vi "test completion complete.vi"(8 "error in (no error)":errorcluster) -> (0 "error out":errorcluster, 3 "body":string)   [LabVIEW 2020, in "MCP Server tests.lvlib"]
doc: "completion/complete (MCP utility completion) in both eras. A legacy initialize (id 731) and a modern server/discover (id 732) declare capabilities.completions {}. completion/complete for the prompt fake_prompt_concatanate_strings is answered with completion.values [], total 0 and hasMore false, legacy (id 733) and modern (id 734, HTTP 200 with resultType complete). completion/complete for a prompt the server does not have (id 735) is answered with the JSON-RPC error -32602 and the request id. The requests are sent with the LabVIEW HTTP Client directly."
uses:
  MCP Server tests.lvlib
  <vilib>/addons/_JKI Toolkits/Caraya/classes/Test/Test.lvclass
  <vilib>/addons/_JKI Toolkits/Caraya/classes/Assert/Assert.lvclass
panel:
  out "lookup error":errorcluster
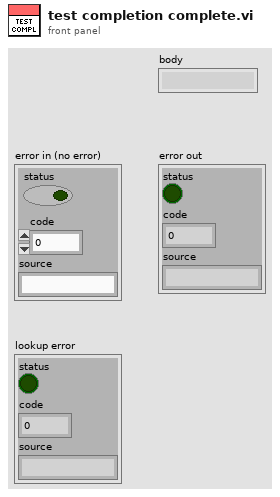
[diagram p1: front panel]
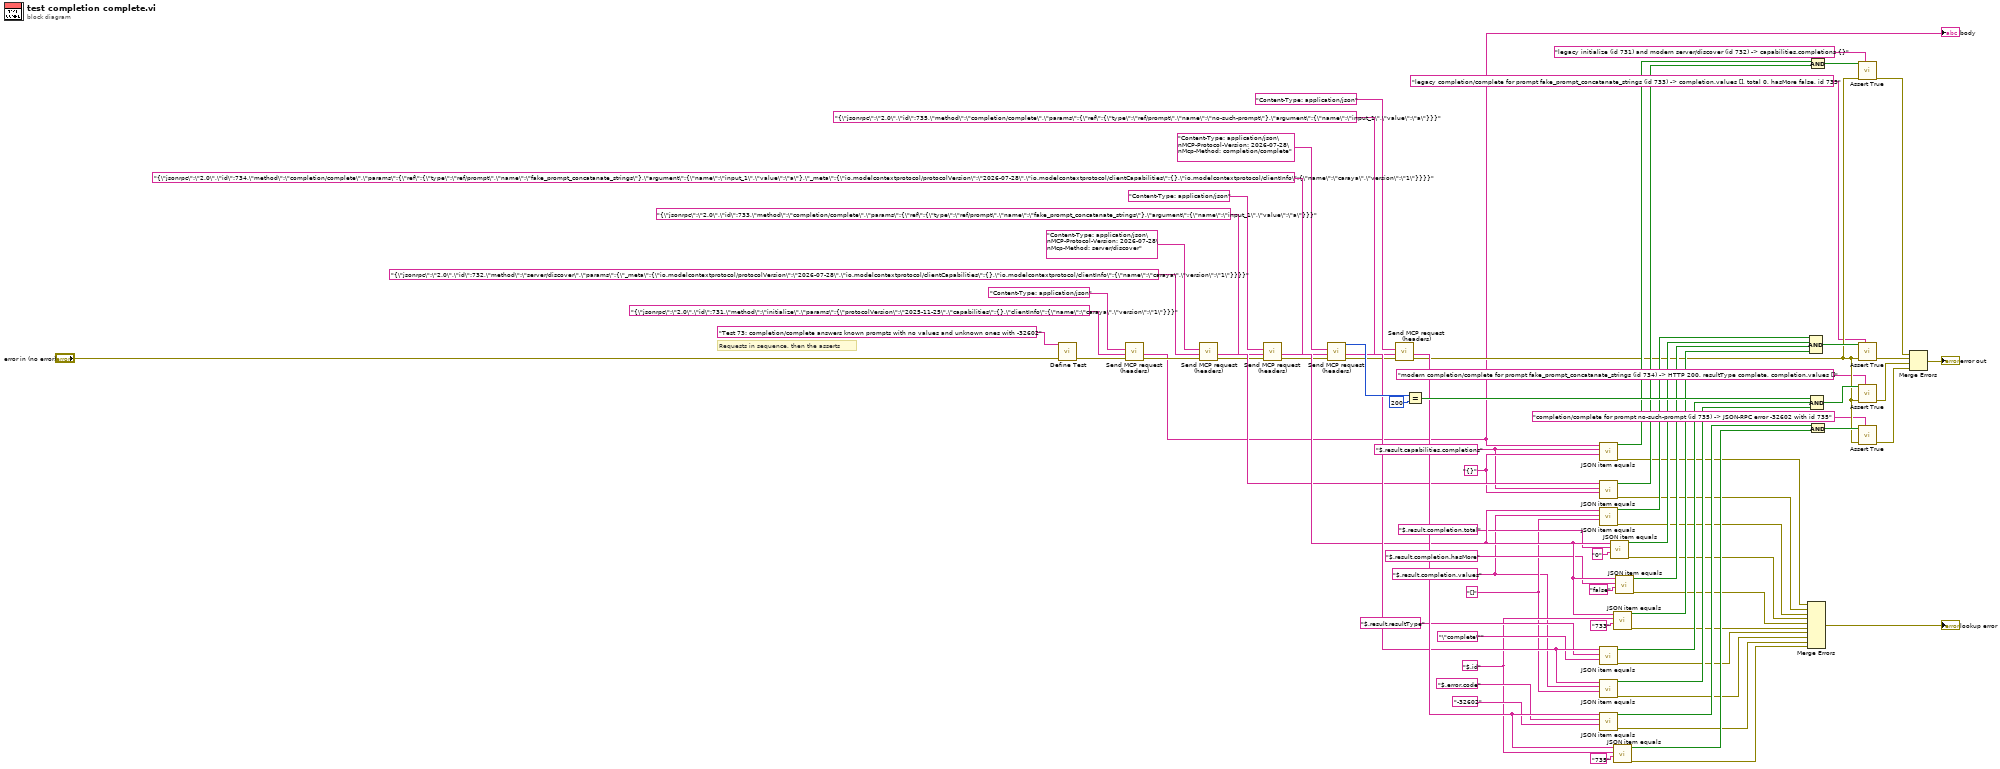
[diagram p0: block diagram]
diagram:
  w24 = "$.id" ("path")
  w19 = "[]" ("expected")
  w18 = "$.result.completion.values" ("path")
  w17 = "{}" ("expected")
  w16 = "$.result.capabilities.completions" ("path")
  # "Requests in sequence, then the asserts"
  n1 = call <vilib>:"Define Test.vi"("error in (no error)"="error in (no error)", "Label (VI Title)"="Test 73: completion/complete answers known prompts with no values and unknown ones with -32602") -> ("error out"=w36:errorcluster)  [unwired: 8 in, 1 out]
  n2 = call "Send MCP request (headers).vi"("error in (no error)"=w36, "request"="{\"jsonrpc\":\"2.0\",\"id\":731,\"method\":\"initialize\",\"params\":{\"protocolVersion\":\"2025-11-25\",\"capabilities\":{},\"clientInfo\":{\"name\":\"caraya\",\"version\":\"1\"}}}", "request headers"="Content-Type: application/json") -> ("error out"=w37:errorcluster, "response"=w2:string)  [unwired: 5 in, 2 out]
  "body" <- w2
  n3 = call "Send MCP request (headers).vi"("error in (no error)"=w37, "request"="{\"jsonrpc\":\"2.0\",\"id\":732,\"method\":\"server/discover\",\"params\":{\"_meta\":{\"io.modelcontextprotocol/protocolVersion\":\"2026-07-28\",\"io.modelcontextprotocol/clientCapabilities\":{},\"io.modelcontextprotocol/clientInfo\":{\"name\":\"caraya\",\"version\":\"1\"}}}}", "request headers"="Content-Type: application/json\nMCP-Protocol-Version: 2026-07-28\nMcp-Method: server/discover") -> ("error out"=w38:errorcluster, "response"=w39:string)  [unwired: 5 in, 2 out]
  n4 = call "Send MCP request (headers).vi"("error in (no error)"=w38, "request"="{\"jsonrpc\":\"2.0\",\"id\":733,\"method\":\"completion/complete\",\"params\":{\"ref\":{\"type\":\"ref/prompt\",\"name\":\"fake_prompt_concatanate_strings\"},\"argument\":{\"name\":\"input_1\",\"value\":\"a\"}}}", "request headers"="Content-Type: application/json") -> ("error out"=w40:errorcluster, "response"=w41:string)  [unwired: 5 in, 2 out]
  n5 = call "Send MCP request (headers).vi"("error in (no error)"=w40, "request"="{\"jsonrpc\":\"2.0\",\"id\":734,\"method\":\"completion/complete\",\"params\":{\"ref\":{\"type\":\"ref/prompt\",\"name\":\"fake_prompt_concatanate_strings\"},\"argument\":{\"name\":\"input_1\",\"value\":\"a\"},\"_meta\":{\"io.modelcontextprotocol/protocolVersion\":\"2026-07-28\",\"io.modelcontextprotocol/clientCapabilities\":{},\"io.modelcontextprotocol/clientInfo\":{\"name\":\"caraya\",\"version\":\"1\"}}}}", "request headers"="Content-Type: application/json\nMCP-Protocol-Version: 2026-07-28\nMcp-Method: completion/complete") -> ("error out"=w42:errorcluster, "response"=w43:string, "status code"=w44:i32)  [unwired: 5 in, 1 out]
  n6 = call "Send MCP request (headers).vi"("error in (no error)"=w42, "request"="{\"jsonrpc\":\"2.0\",\"id\":735,\"method\":\"completion/complete\",\"params\":{\"ref\":{\"type\":\"ref/prompt\",\"name\":\"no-such-prompt\"},\"argument\":{\"name\":\"input_1\",\"value\":\"a\"}}}", "request headers"="Content-Type: application/json") -> ("error out"=w45:errorcluster, "response"=w46:string)  [unwired: 5 in, 2 out]
  n7 = Equal?(x=w44, y=200 ("expected status")) -> (x = y?=w59:bool)
  n8 = call "JSON item equals.vi"("expected"=w17, "path"=w16, "JSON"=w2) -> ("error out"=w47:errorcluster, "equal?"=w48:bool)  [unwired: 6 in, 1 out]
  n9 = call "JSON item equals.vi"("expected"=w17, "path"=w16, "JSON"=w39) -> ("error out"=w49:errorcluster, "equal?"=w50:bool)  [unwired: 6 in, 1 out]
  n10 = call "JSON item equals.vi"("expected"=w19, "path"=w18, "JSON"=w41) -> ("error out"=w51:errorcluster, "equal?"=w52:bool)  [unwired: 6 in, 1 out]
  n11 = call "JSON item equals.vi"("expected"="\"complete\"", "path"="$.result.resultType", "JSON"=w43) -> ("error out"=w60:errorcluster, "equal?"=w61:bool)  [unwired: 6 in, 1 out]
  n12 = call "JSON item equals.vi"("expected"=w19, "path"=w18, "JSON"=w43) -> ("error out"=w62:errorcluster, "equal?"=w63:bool)  [unwired: 6 in, 1 out]
  n13 = call "JSON item equals.vi"("expected"="-32602", "path"="$.error.code", "JSON"=w46) -> ("error out"=w64:errorcluster, "equal?"=w65:bool)  [unwired: 6 in, 1 out]
  n14 = call "JSON item equals.vi"("expected"="0", "path"="$.result.completion.total", "JSON"=w41) -> ("error out"=w53:errorcluster, "equal?"=w54:bool)  [unwired: 6 in, 1 out]
  n15 = call "JSON item equals.vi"("expected"="733", "path"=w24, "JSON"=w41) -> ("error out"=w57:errorcluster, "equal?"=w58:bool)  [unwired: 6 in, 1 out]
  n16 = call "JSON item equals.vi"("expected"="735", "path"=w24, "JSON"=w46) -> ("error out"=w66:errorcluster, "equal?"=w67:bool)  [unwired: 6 in, 1 out]
  n17 = call "JSON item equals.vi"("expected"="false", "path"="$.result.completion.hasMore", "JSON"=w41) -> ("error out"=w55:errorcluster, "equal?"=w56:bool)  [unwired: 6 in, 1 out]
  n18 = Merge Errors(w47, w49, w51, w53, w55, w57, w60, w62, w64, w66) -> (→"lookup error":errorcluster)
  n19 = Compound Arithmetic op=AND(w52, w54, w56, w58) -> (w69:bool)
  n20 = Compound Arithmetic op=AND(w59, w61, w63) -> (w70:bool)
  n21 = Compound Arithmetic op=AND(w48, w50) -> (w68:bool)
  n22 = Compound Arithmetic op=AND(w65, w67) -> (w71:bool)
  n23 = call <vilib>:"Assert True.vi"("Label"="legacy initialize (id 731) and modern server/discover (id 732) -> capabilities.completions {}", "error in (no error)"=w45, "True?"=w68) -> ("error out"=w72:errorcluster)  [unwired: 7 in, 1 out]
  n24 = call <vilib>:"Assert True.vi"("Label"="legacy completion/complete for prompt fake_prompt_concatanate_strings (id 733) -> completion.values [], total 0, hasMore false, id 733", "error in (no error)"=w45, "True?"=w69) -> ("error out"=w73:errorcluster)  [unwired: 7 in, 1 out]
  n25 = call <vilib>:"Assert True.vi"("Label"="modern completion/complete for prompt fake_prompt_concatanate_strings (id 734) -> HTTP 200, resultType complete, completion.values []", "error in (no error)"=w45, "True?"=w70) -> ("error out"=w74:errorcluster)  [unwired: 7 in, 1 out]
  n26 = call <vilib>:"Assert True.vi"("Label"="completion/complete for prompt no-such-prompt (id 735) -> JSON-RPC error -32602 with id 735", "error in (no error)"=w45, "True?"=w71) -> ("error out"=w75:errorcluster)  [unwired: 7 in, 1 out]
  n27 = Merge Errors(w72, w73, w74, w75) -> (→"error out":errorcluster)
